vi "Labview_trieur_balles.vi"(8 "error in (no error)":errorcluster) -> (0 "error out":errorcluster)   [LabVIEW 2018]
uses:
  enum_trieur_balle.ctl
panel:
  in  "delay rotation 6":i32=38000
  in  "delay rotation 5":i32=37000
  in  "delay rotation 4":i32=36000
  in  "delay rotation 3":i32=36500
  in  "delay rotation 2":i32=36000
  in  "delay rotation":i32=39000
  in  "x 2":i32=10000000
  in  "x":i32=10000000
  out "x+1 4":i32
  out "Couleur 4":bool
  out "Cluster 4":T1
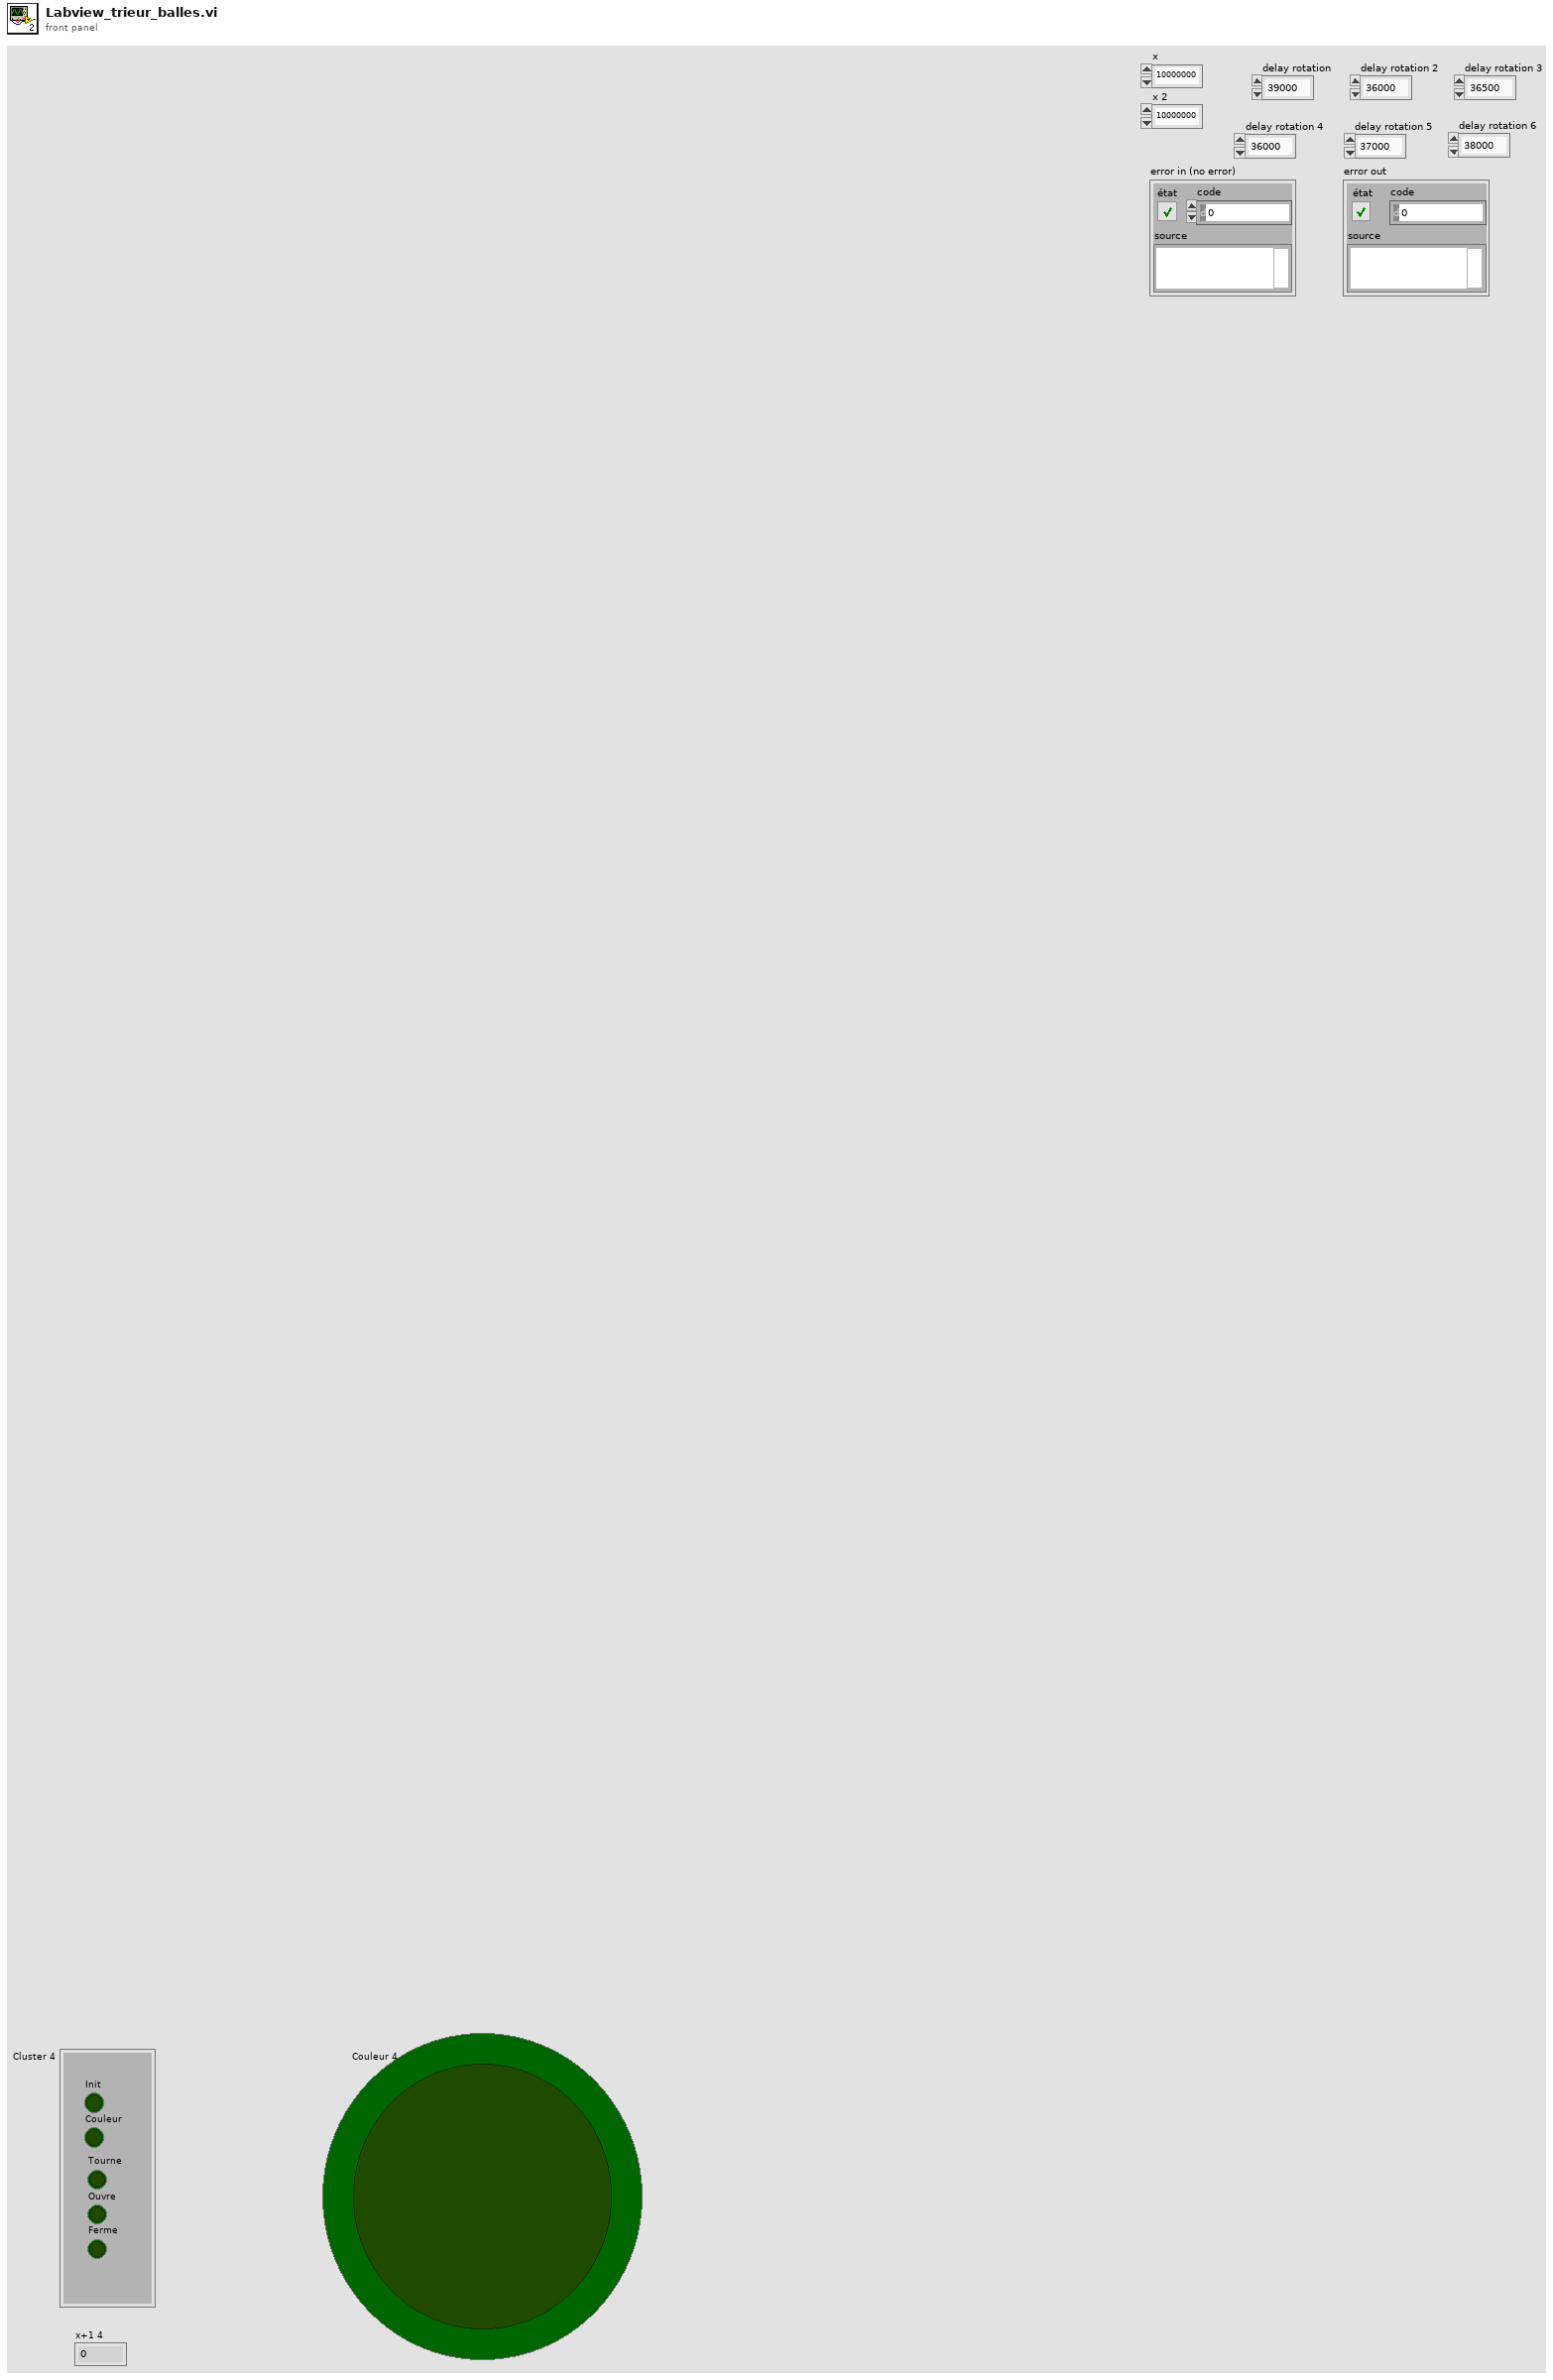
[diagram p1: front panel]
types:
  T1 = cluster{"Init":bool, "Couleur":bool, "Tourne":bool, "Ouvre":bool, "Ferme":bool}
  T2 = typedef "enum_trieur_balle.ctl" = enum16{"Initialisation", "Couleur", "Rotation", "Ouverture", "Fermeture"}
  T3 = cluster{"Booléen":bool, "Booléen 2":bool, "Booléen 3":bool, "Booléen 4":bool, "Booléen 5":bool}
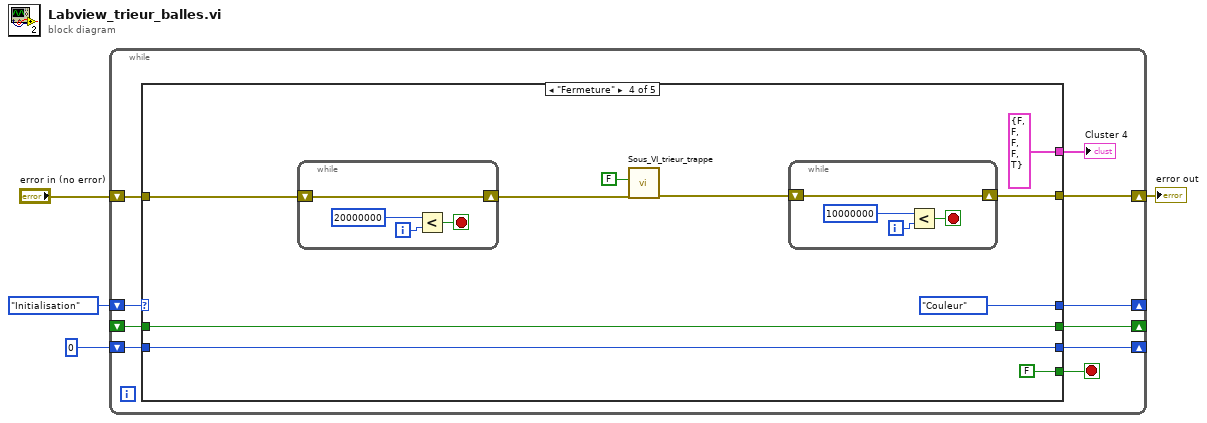
[diagram p0: block diagram]
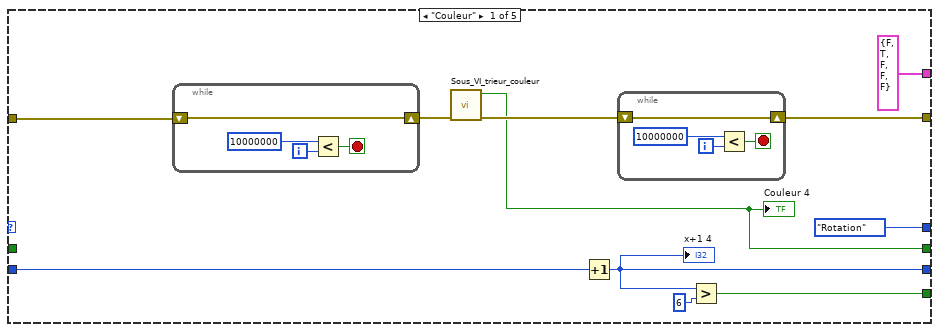
[diagram p2: hidden frame]
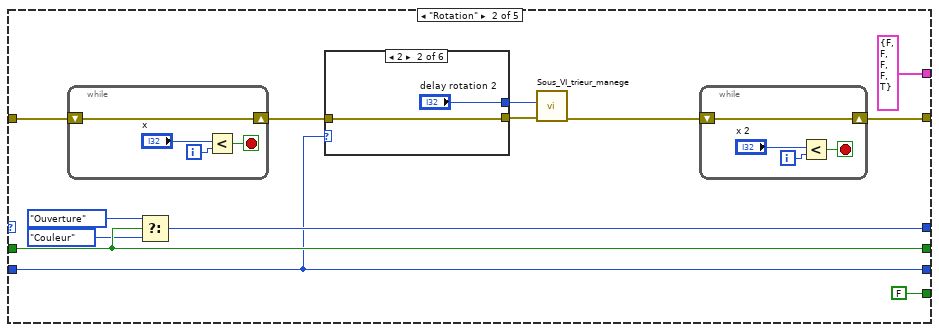
[diagram p3: hidden frame]
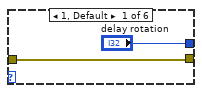
[diagram p4: hidden frame]
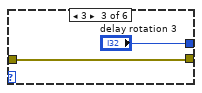
[diagram p5: hidden frame]
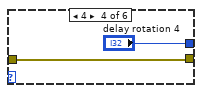
[diagram p6: hidden frame]
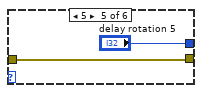
[diagram p7: hidden frame]
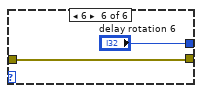
[diagram p8: hidden frame]
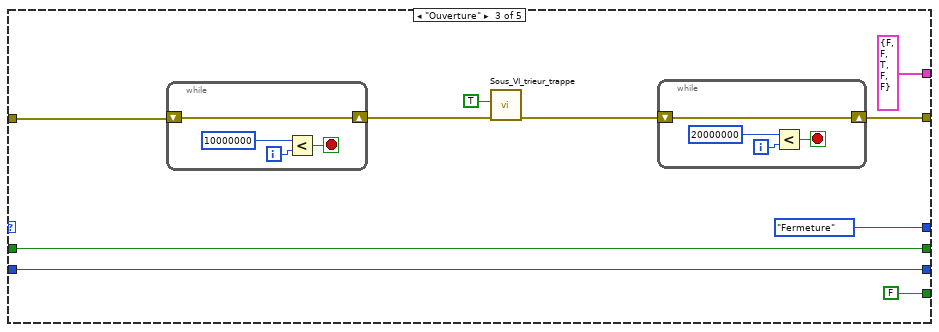
[diagram p9: hidden frame]
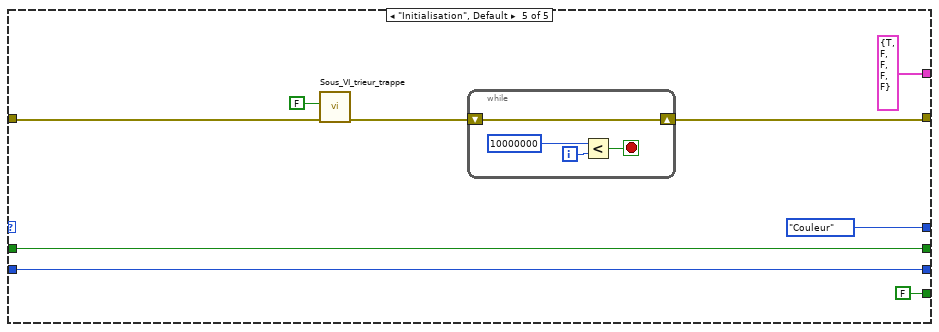
[diagram p10: hidden frame]
diagram:
  n1 = while {
    shift-right: [w10] -> _
    shift-left: enum_trieur_balle."Initialisation" -> [w14]
    shift-right: [w13] -> _
    shift-left: _ -> [w9]
    shift-right: [w11] -> _
    shift-left: 0 -> [w12]
    shift-right: [w5] -> w1
    shift-left: "error in (no error)" -> [w6]
    stop <- w7 stop-if-true
    n2 = case shown="\"Fermeture\"" w14 {
      tunnel: [w15 w44 w76 w93 w108] -> w13
      tunnel: w12 -> [w25 w40 w75 w92 w111]
      tunnel: [w22 w40 w75 w92 w111] -> w11
      tunnel: [w20 FALSE FALSE FALSE FALSE] -> w7
      tunnel: [enum_trieur_balle."Rotation" w45 enum_trieur_balle."Fermeture" enum_trieur_balle."Couleur" enum_trieur_balle."Couleur"] -> w10
      tunnel: w9 -> [_ w44 w76 w93 w108]
      tunnel: [T3 {"Booléen"=FALSE, "Booléen 2"=TRUE, "Booléen 3"=FALSE, "Booléen 4"=FALSE, "Booléen 5"=FALSE} ("Cluster") T3 {"Booléen"=FALSE, "Booléen 2"=FALSE, "Booléen 3"=FALSE, "Booléen 4"=FALSE, "Booléen 5"=TRUE} ("Cluster") T3 {"Booléen"=FALSE, "Booléen 2"=FALSE, "Booléen 3"=TRUE, "Booléen 4"=FALSE, "Booléen 5"=FALSE} ("Cluster") T3 {"Booléen"=FALSE, "Booléen 2"=FALSE, "Booléen 3"=FALSE, "Booléen 4"=FALSE, "Booléen 5"=TRUE} ("Cluster") T3 {"Booléen"=TRUE, "Booléen 2"=FALSE, "Booléen 3"=FALSE, "Booléen 4"=FALSE, "Booléen 5"=FALSE} ("Cluster")] -> w8
      tunnel: w6 -> [w19 w39 w70 w89 w106]
      tunnel: [w16 w36 w68 w86 w104] -> w5
      frame "Couleur" {
        n3 = while {
          shift-right: [w30] -> w18
          shift-left: w19 -> [w30]
          i -> [w33]
          stop <- w31 stop-if-true
          n4 = Less?(x=10000000, y=w33) -> (x < y?=w31:bool)
        }
        n5 = call "Sous_VI_trieur_couleur.vi"("error in (no error)"=w18) -> ("error out"=w17:errorcluster, "Couleur"=w15:bool)  [unwired: 7 in]
        "Couleur 4" <- w15
        n6 = Increment(x=w25) -> (x+1=w22:i32)
        "x+1 4" <- w22
        n7 = while {
          shift-right: [w26] -> w16
          shift-left: w17 -> [w26]
          i -> [w29]
          stop <- w27 stop-if-true
          n8 = Less?(x=10000000, y=w29) -> (x < y?=w27:bool)
        }
        n9 = Greater?(x=w22, y=6) -> (0:w20:bool)
      }
      frame "Rotation" {
        n10 = while {
          shift-right: [w63] -> w38
          shift-left: w39 -> [w63]
          i -> [w66]
          stop <- w65 stop-if-true
          n11 = Less?(x="x", y=w66) -> (x < y?=w65:bool)
        }
        n12 = Select(t=enum_trieur_balle."Ouverture", s=w44, f=enum_trieur_balle."Couleur") -> (s? t:f=w45:T2)
        n13 = case shown="2" w40 {
          tunnel: ["delay rotation" "delay rotation 2" "delay rotation 3" "delay rotation 4" "delay rotation 5" "delay rotation 6"] -> w35
          tunnel: [w51 w53 w55 w57 w59 w61] -> w34
          tunnel: w38 -> [w51 w53 w55 w57 w59 w61]
          frame 1, Default {
          }
          frame 2 {
          }
          frame 3 {
          }
          frame 4 {
          }
          frame 5 {
          }
          frame 6 {
          }
        }
        n14 = call "Sous_VI_trieur_manege.vi"("error in (no error)"=w34, 10:w35) -> ("error out"=w37:errorcluster)  [unwired: 9 in]
        n15 = while {
          shift-right: [w47] -> w36
          shift-left: w37 -> [w47]
          i -> [w50]
          stop <- w49 stop-if-true
          n16 = Less?(x="x 2", y=w50) -> (x < y?=w49:bool)
        }
      }
      frame "Ouverture" {
        n17 = while {
          shift-right: [w81] -> w71
          shift-left: w70 -> [w81]
          i -> [w84]
          stop <- w82 stop-if-true
          n18 = Less?(x=10000000, y=w84) -> (x < y?=w82:bool)
        }
        n19 = call "Sous_VI_trieur_trappe.vi"("error in (no error)"=w71, "Ouvrir"=TRUE) -> ("error out"=w69:errorcluster)  [unwired: 9 in]
        n20 = while {
          shift-right: [w77] -> w68
          shift-left: w69 -> [w77]
          i -> [w80]
          stop <- w78 stop-if-true
          n21 = Less?(x=20000000, y=w80) -> (x < y?=w78:bool)
        }
      }
      frame "Fermeture" {
        n22 = while {
          shift-right: [w99] -> w88
          shift-left: w89 -> [w99]
          i -> [w102]
          stop <- w100 stop-if-true
          n23 = Less?(x=20000000, y=w102) -> (x < y?=w100:bool)
        }
        n24 = call "Sous_VI_trieur_trappe.vi"("error in (no error)"=w88, "Ouvrir"=FALSE) -> ("error out"=w87:errorcluster)  [unwired: 9 in]
        n25 = while {
          shift-right: [w95] -> w86
          shift-left: w87 -> [w95]
          i -> [w98]
          stop <- w96 stop-if-true
          n26 = Less?(x=10000000, y=w98) -> (x < y?=w96:bool)
        }
      }
      frame "Initialisation", Default {
        n27 = call "Sous_VI_trieur_trappe.vi"("error in (no error)"=w106, "Ouvrir"=FALSE) -> ("error out"=w105:errorcluster)  [unwired: 9 in]
        n28 = while {
          shift-right: [w112] -> w104
          shift-left: w105 -> [w112]
          i -> [w115]
          stop <- w113 stop-if-true
          n29 = Less?(x=10000000, y=w115) -> (x < y?=w113:bool)
        }
      }
    }
    "Cluster 4" <- w8
  }
  "error out" <- w1
